vi "Joystick Get Values.vi"(8 "error in (no error)":errorcluster, 11 "Joystick":T1) -> (0 "error out":errorcluster, 1 "Buttons":bool[](array[boolean]), 2 "Axes":dbl[](array[numeric]), 3 "Joystick":T1, 4 "POVs":u8[](array[numeric]), 5 "Touchpads":T2(array[cluster]))   [LabVIEW 2023, in "MrcLib.lvlib"]
doc: "Returns button and scaled axis information for a joystick that you specify."
uses:
  <vilib>/MRC/MrcLib.lvlib
  <vilib>/MRC/Types/WPI_JoystickDeviceEnum.ctl
panel:
  in  "Scaler":i16=32767
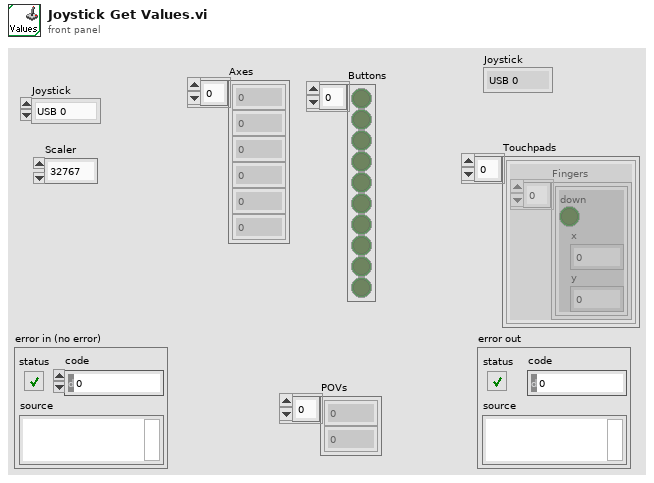
[diagram p1: front panel]
types:
  T1 = typedef "WPI_JoystickDeviceEnum.ctl" = enum16{"USB 0", "USB 1", "USB 2", "USB 3", "USB 4", "USB 5"}
  T2 = cluster{"Fingers":cluster{"down":bool, "x":u16, "y":u16}[]}[]
  T3 = cluster{cluster{"down":bool, "x":u16, "y":u16}[]}
  T4 = typedef "MrcLib.lvlib/MRC_Joysticks.ctl" = cluster{"count":u8, "dummy":cluster{i8, i8, i8, i8, i8, i8, i8}, "joystick 0":cluster{"availablePovs":u8, "povs":cluster{"pov 0":u8, "pov 1":u8, "pov 2":u8, "pov 3":u8, "pov 4":u8, "pov 5":u8, "pov 6":u8, "pov 7":u8}, "availableAxes":u16, "axes":cluster{"axis 0":i16, "axis 1":i16, "axis 2":i16, "axis 3":i16, "axis 4":i16, "axis 5":i16, "axis 6":i16, "axis 7":i16, "axis 8":i16, "axis 9":i16, "axis 10":i16, "axis 11":i16}, "availableButtons":u64, "buttons":u64, "touchPads":cluster{"touchPadCount":u8, "touchpad 1":cluster{"count":u8, "finger 1":cluster{"down":u8, "x":u16, "y":u16}, "finger 2":cluster{"down":u8, "x":u16, "y":u16}}, "touchpad 2":cluster{"count":u8, "finger 1":cluster{"down":u8, "x":u16, "y":u16}, "finger 2":cluster{"down":u8, "x":u16, "y":u16}}}}, "joystick 1":cluster{"availablePovs":u8, "povs":cluster{"pov 0":u8, "pov 1":u8, "pov 2":u8, "pov 3":u8, "pov 4":u8, "pov 5":u8, "pov 6":u8, "pov 7":u8}, "availableAxes":u16, "axes":cluster{"axis 0":i16, "axis 1":i16, "axis 2":i16, "axis 3":i16, "axis 4":i16, "axis 5":i16, "axis 6":i16, "axis 7":i16, "axis 8":i16, "axis 9":i16, "axis 10":i16, "axis 11":i16}, "availableButtons":u64, "buttons":u64, "touchPads":cluster{"touchPadCount":u8, "touchpad 1":cluster{"count":u8, "finger 1":cluster{"down":u8, "x":u16, "y":u16}, "finger 2":cluster{"down":u8, "x":u16, "y":u16}}, "touchpad 2":cluster{"count":u8, "finger 1":cluster{"down":u8, "x":u16, "y":u16}, "finger 2":cluster{"down":u8, "x":u16, "y":u16}}}}, "joystick 2":cluster{"availablePovs":u8, "povs":cluster{"pov 0":u8, "pov 1":u8, "pov 2":u8, "pov 3":u8, "pov 4":u8, "pov 5":u8, "pov 6":u8, "pov 7":u8}, "availableAxes":u16, "axes":cluster{"axis 0":i16, "axis 1":i16, "axis 2":i16, "axis 3":i16, "axis 4":i16, "axis 5":i16, "axis 6":i16, "axis 7":i16, "axis 8":i16, "axis 9":i16, "axis 10":i16, "axis 11":i16}, "availableButtons":u64, "buttons":u64, "touchPads":cluster{"touchPadCount":u8, "touchpad 1":cluster{"count":u8, "finger 1":cluster{"down":u8, "x":u16, "y":u16}, "finger 2":cluster{"down":u8, "x":u16, "y":u16}}, "touchpad 2":cluster{"count":u8, "finger 1":cluster{"down":u8, "x":u16, "y":u16}, "finger 2":cluster{"down":u8, "x":u16, "y":u16}}}}, "joystick 3":cluster{"availablePovs":u8, "povs":cluster{"pov 0":u8, "pov 1":u8, "pov 2":u8, "pov 3":u8, "pov 4":u8, "pov 5":u8, "pov 6":u8, "pov 7":u8}, "availableAxes":u16, "axes":cluster{"axis 0":i16, "axis 1":i16, "axis 2":i16, "axis 3":i16, "axis 4":i16, "axis 5":i16, "axis 6":i16, "axis 7":i16, "axis 8":i16, "axis 9":i16, "axis 10":i16, "axis 11":i16}, "availableButtons":u64, "buttons":u64, "touchPads":cluster{"touchPadCount":u8, "touchpad 1":cluster{"count":u8, "finger 1":cluster{"down":u8, "x":u16, "y":u16}, "finger 2":cluster{"down":u8, "x":u16, "y":u16}}, "touchpad 2":cluster{"count":u8, "finger 1":cluster{"down":u8, "x":u16, "y":u16}, "finger 2":cluster{"down":u8, "x":u16, "y":u16}}}}, "joystick 4":cluster{"availablePovs":u8, "povs":cluster{"pov 0":u8, "pov 1":u8, "pov 2":u8, "pov 3":u8, "pov 4":u8, "pov 5":u8, "pov 6":u8, "pov 7":u8}, "availableAxes":u16, "axes":cluster{"axis 0":i16, "axis 1":i16, "axis 2":i16, "axis 3":i16, "axis 4":i16, "axis 5":i16, "axis 6":i16, "axis 7":i16, "axis 8":i16, "axis 9":i16, "axis 10":i16, "axis 11":i16}, "availableButtons":u64, "buttons":u64, "touchPads":cluster{"touchPadCount":u8, "touchpad 1":cluster{"count":u8, "finger 1":cluster{"down":u8, "x":u16, "y":u16}, "finger 2":cluster{"down":u8, "x":u16, "y":u16}}, "touchpad 2":cluster{"count":u8, "finger 1":cluster{"down":u8, "x":u16, "y":u16}, "finger 2":cluster{"down":u8, "x":u16, "y":u16}}}}, "joystick 5":cluster{"availablePovs":u8, "povs":cluster{"pov 0":u8, "pov 1":u8, "pov 2":u8, "pov 3":u8, "pov 4":u8, "pov 5":u8, "pov 6":u8, "pov 7":u8}, "availableAxes":u16, "axes":cluster{"axis 0":i16, "axis 1":i16, "axis 2":i16, "axis 3":i16, "axis 4":i16, "axis 5":i16, "axis 6":i16, "axis 7":i16, "axis 8":i16, "axis 9":i16, "axis 10":i16, "axis 11":i16}, "availableButtons":u64, "buttons":u64, "touchPads":cluster{"touchPadCount":u8, "touchpad 1":cluster{"count":u8, "finger 1":cluster{"down":u8, "x":u16, "y":u16}, "finger 2":cluster{"down":u8, "x":u16, "y":u16}}, "touchpad 2":cluster{"count":u8, "finger 1":cluster{"down":u8, "x":u16, "y":u16}, "finger 2":cluster{"down":u8, "x":u16, "y":u16}}}}}
  T5 = cluster{"availablePovs":u8, "povs":cluster{"pov 0":u8, "pov 1":u8, "pov 2":u8, "pov 3":u8, "pov 4":u8, "pov 5":u8, "pov 6":u8, "pov 7":u8}, "availableAxes":u16, "axes":cluster{"axis 0":i16, "axis 1":i16, "axis 2":i16, "axis 3":i16, "axis 4":i16, "axis 5":i16, "axis 6":i16, "axis 7":i16, "axis 8":i16, "axis 9":i16, "axis 10":i16, "axis 11":i16}, "availableButtons":u64, "buttons":u64, "touchPads":cluster{"touchPadCount":u8, "touchpad 1":cluster{"count":u8, "finger 1":cluster{"down":u8, "x":u16, "y":u16}, "finger 2":cluster{"down":u8, "x":u16, "y":u16}}, "touchpad 2":cluster{"count":u8, "finger 1":cluster{"down":u8, "x":u16, "y":u16}, "finger 2":cluster{"down":u8, "x":u16, "y":u16}}}}
  T6 = cluster{"pov 0":u8, "pov 1":u8, "pov 2":u8, "pov 3":u8, "pov 4":u8, "pov 5":u8, "pov 6":u8, "pov 7":u8}
  T7 = cluster{"axis 0":i16, "axis 1":i16, "axis 2":i16, "axis 3":i16, "axis 4":i16, "axis 5":i16, "axis 6":i16, "axis 7":i16, "axis 8":i16, "axis 9":i16, "axis 10":i16, "axis 11":i16}
  T8 = cluster{"touchPadCount":u8, "touchpad 1":cluster{"count":u8, "finger 1":cluster{"down":u8, "x":u16, "y":u16}, "finger 2":cluster{"down":u8, "x":u16, "y":u16}}, "touchpad 2":cluster{"count":u8, "finger 1":cluster{"down":u8, "x":u16, "y":u16}, "finger 2":cluster{"down":u8, "x":u16, "y":u16}}}
  T9 = cluster{"count":u8, "finger 1":cluster{"down":u8, "x":u16, "y":u16}, "finger 2":cluster{"down":u8, "x":u16, "y":u16}}
  T10 = cluster{"count":u8, "finger 1":cluster{"down":u8, "x":u16, "y":u16}, "finger 2":cluster{"down":u8, "x":u16, "y":u16}}[]
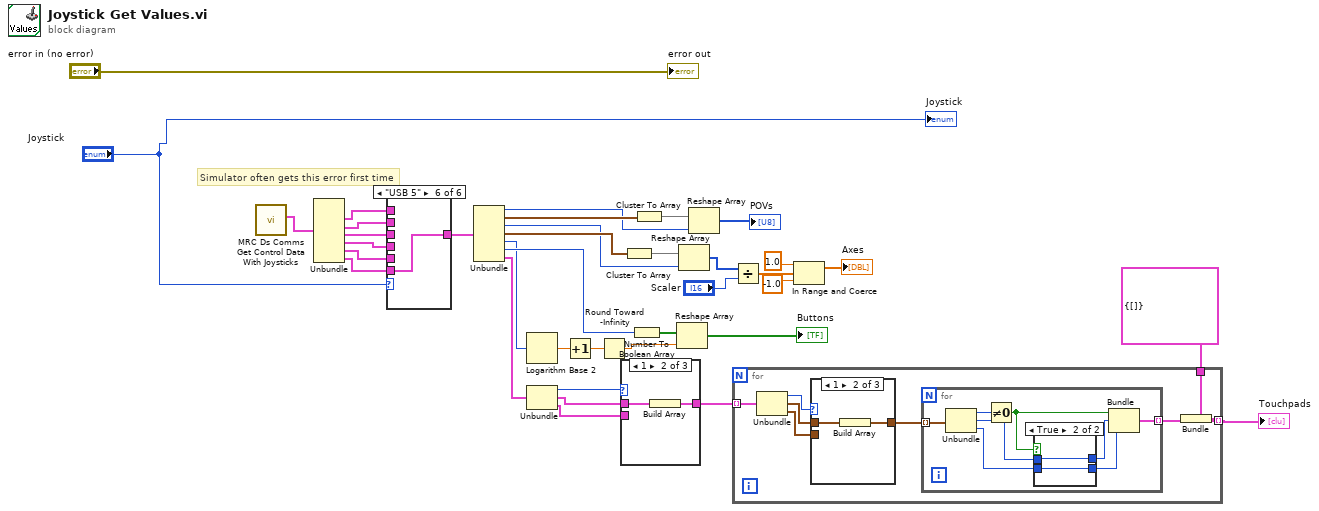
[diagram p0: block diagram]
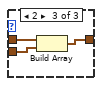
[diagram p4: hidden frame]
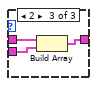
[diagram p6: hidden frame]
diagram:
  # "Simulator often gets this error first time"
  n1 = call <vilib>:"MRC Ds Comms Get Control Data With Joysticks.vi"() -> ("joystickData out"=w33:T4)  [unwired: 9 in, 2 out]
  n2 = Unbundle(w33) -> ("joystick 0"=w32:T5, "joystick 1"=w31:T5, "joystick 2"=w30:T5, "joystick 3"=w29:T5, "joystick 4"=w28:T5, "joystick 5"=w27:T5)  [unwired: 2 out]
  n3 = case shown="\"USB 5\"" "Joystick" {
    tunnel: [w38 w39 w40 w41 w42 w43] -> w26
    tunnel: w32 -> [w38 _ _ _ _ _]
    tunnel: w31 -> [_ w39 _ _ _ _]
    tunnel: w30 -> [_ _ w40 _ _ _]
    tunnel: w29 -> [_ _ _ w41 _ _]
    tunnel: w28 -> [_ _ _ _ w42 _]
    tunnel: w27 -> [_ _ _ _ _ w43]
    frame "USB 0", Default {
    }
    frame "USB 1" {
    }
    frame "USB 2" {
    }
    frame "USB 3" {
    }
    frame "USB 4" {
    }
    frame "USB 5" {
    }
  }
  n4 = Unbundle(w26) -> ("availablePovs"=w23:u8, "povs"=w25:T6, "availableAxes"=w19:u16, "axes"=w20:T7, "availableButtons"=w4:u64, "buttons"=w15:u64, "touchPads"=w13:T8)
  n5 = Logarithm Base 2(1:w4) -> (0:w3:dbl)
  n6 = Unbundle(w13) -> ("touchPadCount"=w12:u8, "touchpad 1"=w11:T9, "touchpad 2"=w10:T9)
  n7 = Increment(x=w3) -> (x+1=w2:dbl)
  n8 = Round Toward -Infinity(1:w2) -> (0:w1:dbl)
  n9 = case shown="1" w12 {
    tunnel: w11 -> [_ w45 w48]
    tunnel: w10 -> [_ _ w47]
    tunnel: [_ w44 w46] -> w9
    frame 0, Default {
    }
    frame 1 {
      n10 = Build Array(w45) -> (w44:T10)
    }
    frame 2 {
      n11 = Build Array(w48, w47) -> (w46:T10)
    }
  }
  n12 = Cluster To Array(cluster=w20) -> (array=w21:i16[])
  n13 = Number To Boolean Array(number=w15) -> (Boolean array=w16:bool[])
  n14 = Cluster To Array(cluster=w25) -> (array=w24:u8[])
  n15 = Reshape Array(w16, w1) -> (→"Buttons":bool[])
  n16 = Reshape Array(w21, w19) -> (w18:i16[])
  n17 = Reshape Array(w24, w23) -> (→"POVs":u8[])
  n18 = Divide(x=w18, y="Scaler") -> (x/y=w37:dbl[])
  n19 = for {
    tunnel: w9 -> [w56] mode=indexing
    tunnel: [w50] -> w7 mode=indexing
    tunnel: T3 {[]} -> [w49]
    n20 = Unbundle(w56) -> ("count"=w55:u8, "finger 1"=w54:cluster{"down":u8, "x":u16, "y":u16}, "finger 2"=w53:cluster{"down":u8, "x":u16, "y":u16})
    n21 = case shown="1" w55 {
      tunnel: w54 -> [_ w68 w71]
      tunnel: w53 -> [_ _ w70]
      tunnel: [_ w67 w69] -> w52
      frame 0, Default {
      }
      frame 1 {
        n22 = Build Array(w68) -> (w67:cluster{"down":u8, "x":u16, "y":u16}[])
      }
      frame 2 {
        n23 = Build Array(w71, w70) -> (w69:cluster{"down":u8, "x":u16, "y":u16}[])
      }
    }
    n24 = for {
      tunnel: w52 -> [w64] mode=indexing
      tunnel: [w62] -> w51 mode=indexing
      n25 = Unbundle(w64) -> ("down"=w63:u8, "x"=w60:u16, "y"=w59:u16)
      n26 = Not Equal To 0?(x=w63) -> (x != 0?=w61:bool)
      n27 = case shown="True" w61 {
        tunnel: w60 -> [_ w66]
        tunnel: w59 -> [_ w65]
        tunnel: [_ w66] -> w58
        tunnel: [_ w65] -> w57
        frame False {
        }
        frame True {
        }
      }
      n28 = Bundle(w61, "x"=w58, "y"=w57) -> (w62:cluster{bool, "x":u16, "y":u16})  [unwired: 1 in]
    }
    n29 = Bundle(cluster=w49, w51) -> (w50:T3)
  }
  "Touchpads" <- w7
  n30 = In Range and Coerce(upper limit=1.0, x=w37, lower limit=-1.0) -> (coerced(x)=→"Axes":dbl[])  [unwired: 1 out]
  "error out" <- "error in (no error)"
  "Joystick" <- "Joystick"
